vi "StartQ0Stream.vi"(8 "error in (no error)":errorcluster, 9 "overwrite":bool, 10 "stream path":path, 11 "Scope5761 in":refnum<class "Scope5782_six_channel.lvclass">) -> (0 "error out":errorcluster, 3 "Scope5761 out":refnum<class "Scope5782_six_channel.lvclass">)   [LabVIEW 2025, in "Scope5782_six_channel.lvclass"]
uses:
  Scope5782_six_channel.lvclass
  FileStream/DumpFileAction.ctl
  Scope5782_six_channel.lvclass/Scope5782_six_channel.ctl
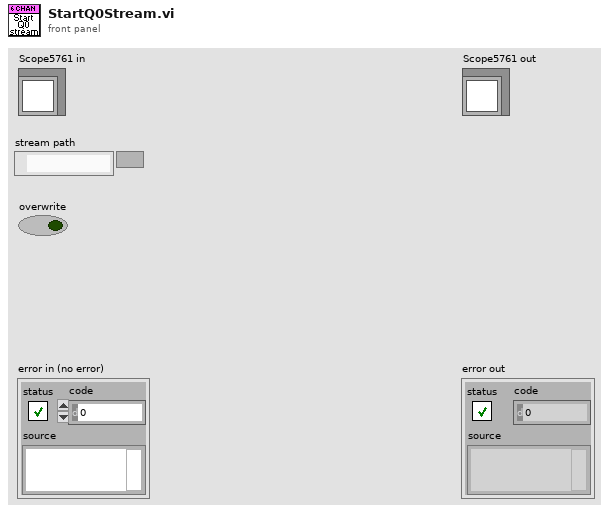
[diagram p1: front panel]
types:
  T1 = typedef "DumpFileAction.ctl" = enum16{"StartNew", "StartAppend", "Data", "Close"}
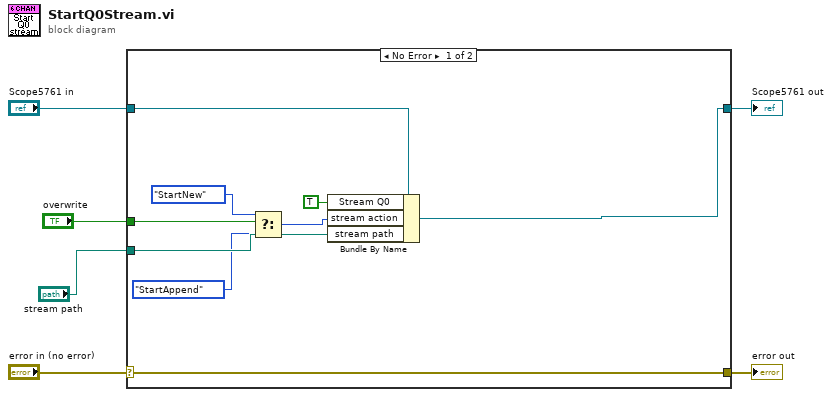
[diagram p0: block diagram]
diagram:
  n1 = case shown="No Error" "error in (no error)" {
    selector: "error in (no error)" -> [w15 w17]
    tunnel: [w15 w17] -> w5
    tunnel: [w7 w16] -> w3
    tunnel: "Scope5761 in" -> [w8 w16]
    tunnel: "stream path" -> [w13 _]
    tunnel: "overwrite" -> [w9 _]
    frame No Error {
      n2 = Select(t=DumpFileAction."StartNew" ("stream action"), s=w9, f=DumpFileAction."StartAppend" ("stream action")) -> (s? t:f=w11:T1)
      n3 = Bundle By Name(cluster=w8, "Stream Q0"=TRUE, "stream action"=w11, "stream path"=w13) -> (w7:refnum<class "Scope5782_six_channel.lvclass">)
    }
    frame Error {
    }
  }
  "error out" <- w5
  "Scope5761 out" <- w3
